vi "Read U8.vi"(8 "error in (no error)":errorcluster, 11 "Event in":refnum<class "Event U8.lvclass">) -> (0 "error out":errorcluster, 2 "U8":u8, 3 "Event out":refnum<class "Event U8.lvclass">)   [LabVIEW 2023, in "MVC Actors.lvlib" / "Event U8.lvclass"]
uses:
  Event U8.lvclass
  Event U8.lvclass/Event U8.ctl
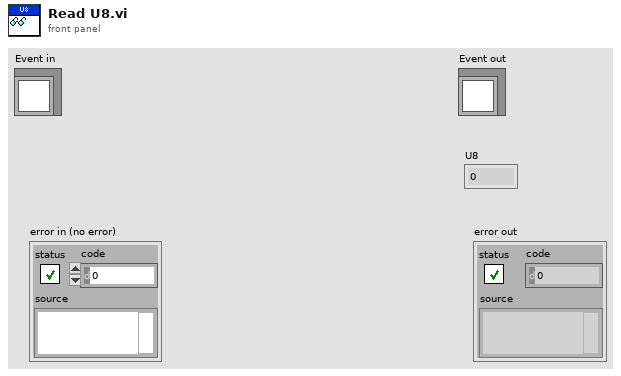
[diagram p1: front panel]
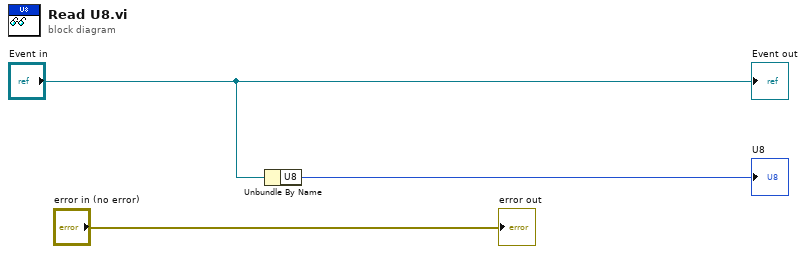
[diagram p0: block diagram]
diagram:
  n1 = Unbundle By Name("Event in") -> ("U8"=→"U8":u8)
  "Event out" <- "Event in"
  "error out" <- "error in (no error)"
